vi "Cmd_Connect.vi"(8 "error in (no error)":errorcluster) -> (0 "error out":errorcluster, 2 "Enum":T1, 3 "Refnum out":refnum<k21>)   [LabVIEW 2025]
uses:
  vi/thresholds.ctl
  Command.ctl
  RT_Cmd.ctl
  states.ctl
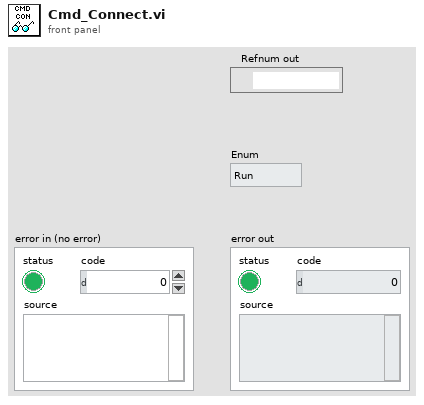
[diagram p1: front panel]
types:
  T1 = typedef "states.ctl" = enum16{"Run", "Connect"}
  T2 = typedef "RT_Cmd.ctl" = cluster{"command":T3, "parameters":T4}
  T3 = typedef "Command.ctl" = enum16{"threshold_config", "manual_trigger", "stop"}
  T4 = typedef "thresholds.ctl" = cluster{"Thr_X":i16, "Thr_Y":i16, "Thr_Z":i16}
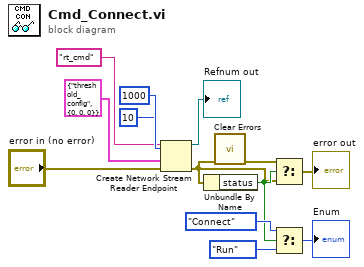
[diagram p0: block diagram]
diagram:
  n1 = Create Network Stream Reader Endpoint(5:1000 ("timeout in ms (-1)"), 7:10 ("reader buffer size"), 8:"error in (no error)", 9:T2 {"command"=enum."threshold_config", "parameters"={"Thr_X"=0, "Thr_Y"=0, "Thr_Z"=0}} ("data"), 11:"rt_cmd" ("reader name")) -> (0:w6:errorcluster, 3:→"Refnum out":refnum<k21>)  [unwired: 2 in]
  n2 = Unbundle By Name(w6) -> ("status"=w7:bool)
  n3 = call <vilib>:"Clear Errors.vi"("error in (no error)"=w6) -> ("error out"=w5:errorcluster)  [unwired: 5 in, 1 out]
  n4 = Select(t=w5, s=w7, f=w6) -> (s? t:f=→"error out":errorcluster)
  n5 = Select(t=states."Connect", s=w7, f=states."Run") -> (s? t:f=→"Enum":T1)
